vi "LinearPlntInvFF_Reset_Initial.vi"(10 "initialState":T1, 11 "Input Linear Plant Inv FF":T2) -> (0 "Size Coerced":bool, 3 "Output Linear Plant Inv FF":T2)   [LabVIEW 2019, in "Trajectory_Library.lvlib"]
doc: "Resets the feedforward with a specified initial state vector.\n \nInputs:\n - LinearPlntInversionFF -- system data cluster\n - initialState -- The initial state vector.\n\nOutputs:\n - outLinearPlntInversionFF -- updated system data cluster\n - sizeCoerced -- If TRUE, an error occured."
uses:
  Trajectory_Library.lvlib
  <vilib>/Analysis/Matrix/Datatypes/RealMatrix.ctl
  <vilib>/Analysis/Matrix/NI_Matrix.lvlib
  TypeDef/LINEAR_PLANT_INV_FF.ctl
panel:
  # "<States,1>"
  # "<Inputs,1>"
  # "<States,Inputs>"
  # "<States,States>"
  # "<States,1>"
  # "<Inputs,1>"
  # "<States,Inputs>"
  # "<States,States>"
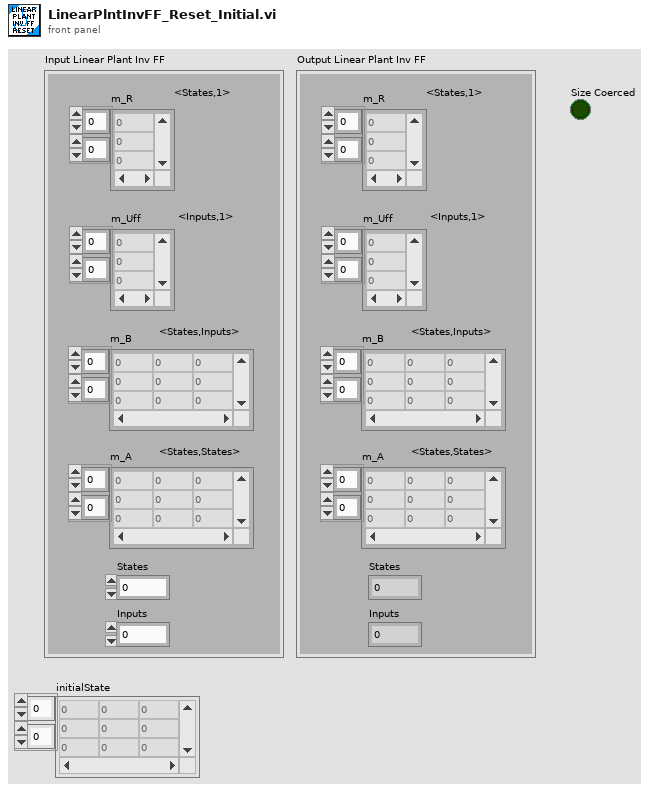
[diagram p1: front panel]
types:
  T1 = typedef "NI_Matrix.lvlib/RealMatrix.ctl" = dbl[][]
  T2 = typedef "Trajectory_Library.lvlib/LINEAR_PLANT_INV_FF.ctl" = cluster{"m_R":T1, "m_Uff":T1, "m_B":T1, "m_A":T1, "States":i32, "Inputs":i32}
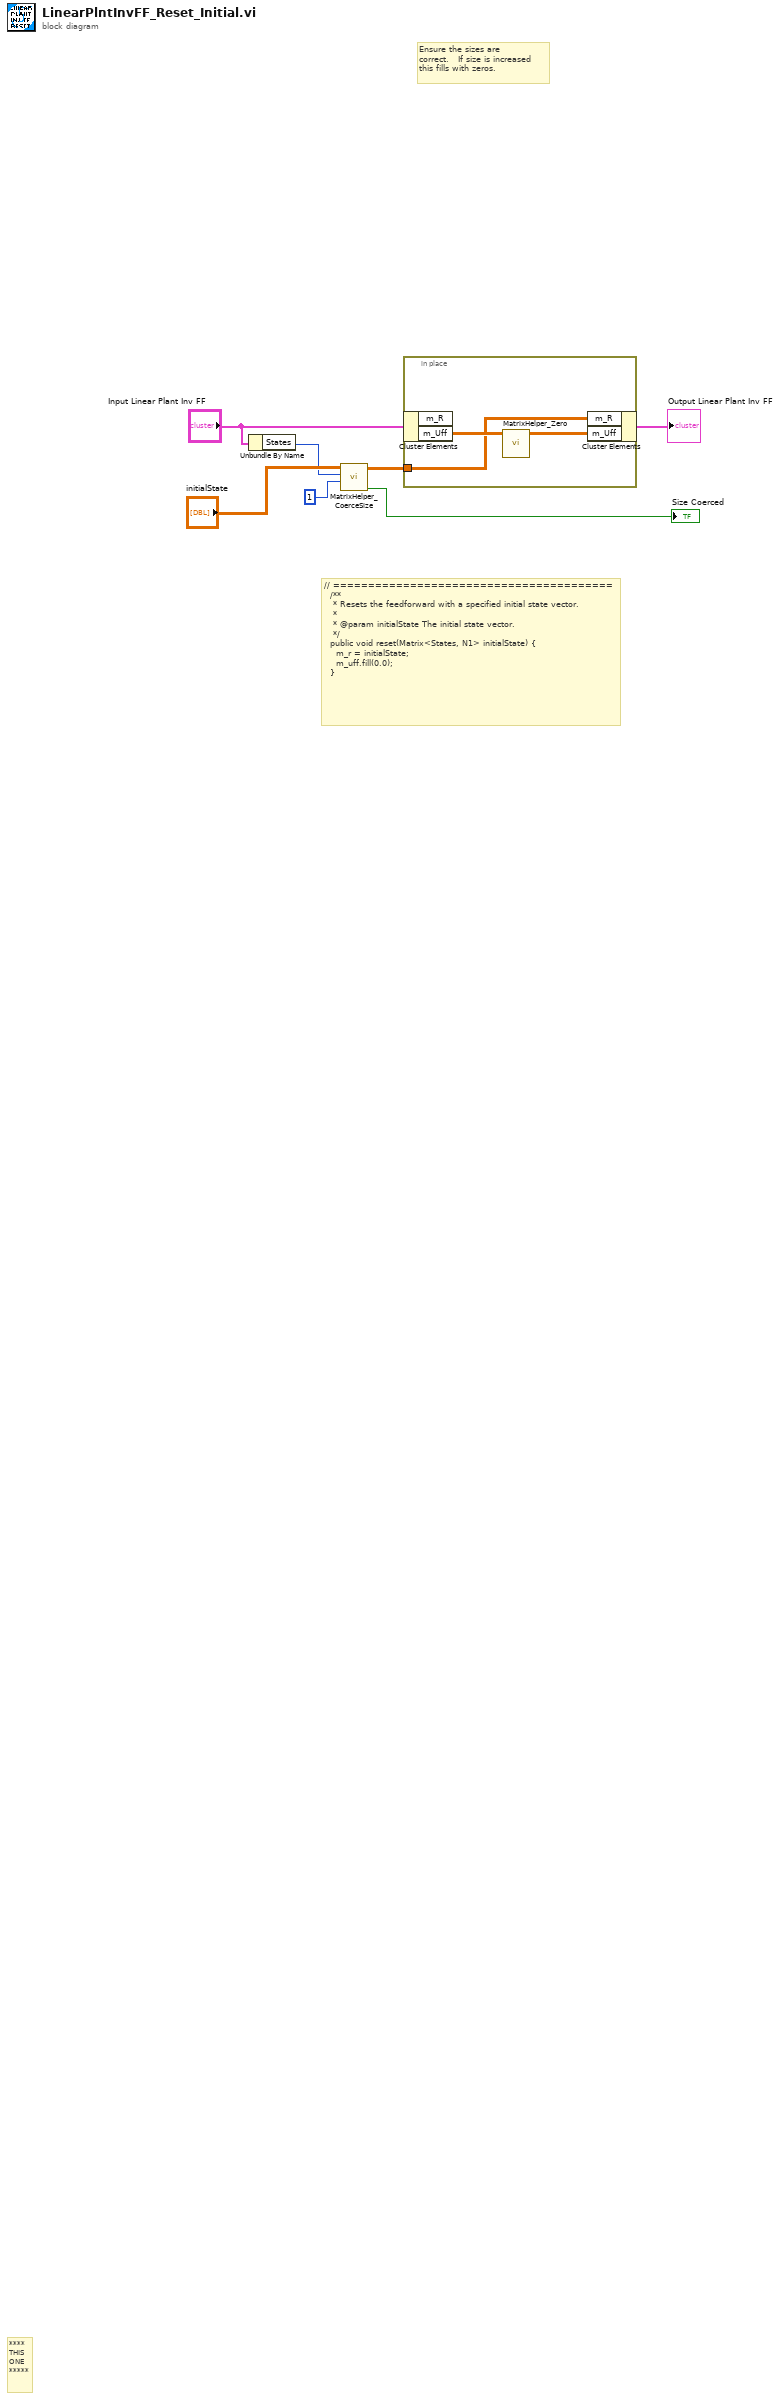
[diagram p0: block diagram]
diagram:
  # "// ========================================\n  /**\n   * Resets the feedforward with a specified initial state vector.\n   *\n   * @param initialState The initial state vector.\n   */\n  public void reset(Matrix<States, N1> initialState) {\n    m_r = initialState;\n    m_uff.fill(0.0);\n  }"
  # "Ensure the sizes are\ncorrect.   If size is increased \nthis fills with zeros."
  # "****\nTHIS\nONE\n*****"
  n1 = Unbundle By Name("Input Linear Plant Inv FF") -> ("States"=w3:i32)
  n2 = call "MatrixHelper_CoerceSize.vi"("Columns"=1, "Rows"=w3, "input matrix"="initialState") -> ("Coerced"=→"Size Coerced":bool, "output matrix"=w5:T1)  [unwired: 7 in]
  n3 = in-place {
    in-place-border: w5 -> [w8]
    n4 = in-place-cluster #1("Input Linear Plant Inv FF") -> ("m_Uff"=w10:T1)  [unwired: 1 out]
    n5 = call "MatrixHelper_Zero.vi"("input matrix"=w10) -> ("output matrix"=w9:T1)  [unwired: 10 in]
    n6 = in-place-cluster #1("m_R"=w8, "m_Uff"=w9) -> (→"Output Linear Plant Inv FF":T2)
  }
